vi "CSE - Variables Writer ID.vi"(6 "set (F)":bool, 8 "error in":errorcluster, 10 "writer ID in":u32, 11 "CSE RefNum":T1) -> (0 "error out":errorcluster, 2 "writer ID out":u32, 3 "dup CSE RefNum":T1)   [LabVIEW 2021]
doc: "Use this VI to preset the <b>writer ID</b> used by the given CSE Instance for writing to variables during execution. The <b>writer ID</b> can also be modified using the <b>vwrid(wrid)</b> function in an expression/script. Refer to the VI help for more details.\n\n<b>CSE RefNum</b> must contain a reference to a CSE instance context.\n\n<b>writer ID in</b> control specifies the value to preset.\n\n<b>writer ID out</b> indicator returns the actual value.\n\n<b>set (F)</b> control defines the action to perform. If FALSE (default), the VI returns the actual writer ID; otherwise, it sets a new value from the <b>writer ID in</b> control.\n\n::: CalcExpress Toolkit :::\nCopyright (c) 2000-2026 Konstantin Shifershteyn. All rights reserved."
uses:
  CSE Instance RefNum.ctl
  cersrc/celveng32.dll
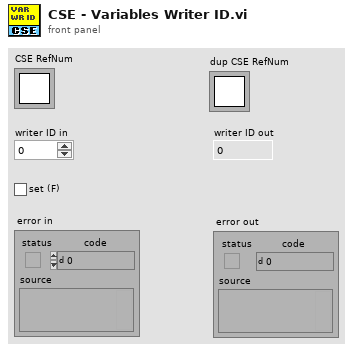
[diagram p1: front panel]
types:
  T1 = typedef "CSE Instance RefNum.ctl" = refnum<k1>
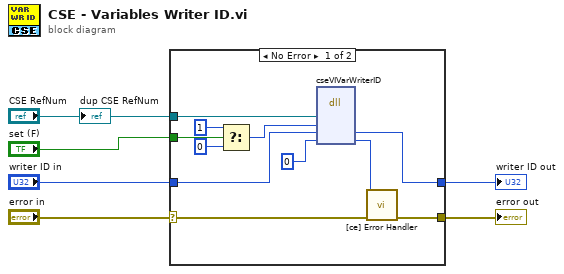
[diagram p0: block diagram]
diagram:
  n1 = case shown="No Error" "error in" {
    selector: "error in" -> [w14 w19]
    tunnel: "CSE RefNum" -> [w17 _]
    tunnel: [w13 w19] -> w4
    tunnel: "set (F)" -> [w9 _]
    tunnel: "writer ID in" -> [w8 w18]
    tunnel: [w7 w18] -> w1
    frame No Error {
      n2 = Select(t=1, s=w9, f=0) -> (s? t:f=w12:i32)
      n3 = dll-call lib="C:/LV Projects/CalcExpress 40 LV2021/vi.lib/addons/CalcExpress/cersrc/celveng*.dll" fn="cseVIVarWriterID"("iCSE"=w17, "cmd"=w12, "writerID"=w8, "errStat"=0) -> ("writerID"=w7:u32, "errStat"=w15:i32)  [unwired: 6 in, 2 out]
      n4 = call "[ce] Error Handler.vi"("error in"=w14, "error code"=w15) -> ("error out"=w13:errorcluster)  [unwired: 8 in, 1 out]
    }
    frame Error {
    }
  }
  "error out" <- w4
  "writer ID out" <- w1
  "dup CSE RefNum" <- "CSE RefNum"
